vi "Local Client.vi"(6 "timeout (ms) [500]":i32=500, 8 "error in (no error)":errorcluster, 9 "params":variant, 10 "Command in":variant, 11 "Instrument in":refnum<class "Instrument.lvclass">) -> (0 "error out":errorcluster, 1 "Data out":variant, 2 "Command out":string, 3 "Instrument out":refnum<class "Instrument.lvclass">)   [LabVIEW 2019, in "Instrument.lvlib" / "Instrument.lvclass"]
doc: "Send a message to a local Instrument process. This VI is basically a wrapper for Instrument.sendMessageToProcess.vi with a mailbox to receive responses.\n\n<b>Command in</b> is a String. Conversion from Enum needs to be handled before calling this method (Use \"Enum to String.vi\")\n\n<b>Data in</b> is a Variant containing your data payload.\n\n<b>Data out</b> is a Variant."
uses:
  Instrument.lvclass
  c6c297fa-ccfe-4267-9780-fc415f7827cf.vi
  Instrument.sendMessageToProcess (variant).vi
  <vilib>/Utility/Data Type/Get Type Information.vi
  <vilib>/Utility/Data Type/Get Numeric Information.vi
  <userlib>/_OpenG.lib/lvdata/lvdata.llb/Unwrap VVariant__ogtk.vi
panel:
  # "Local Client.vi"
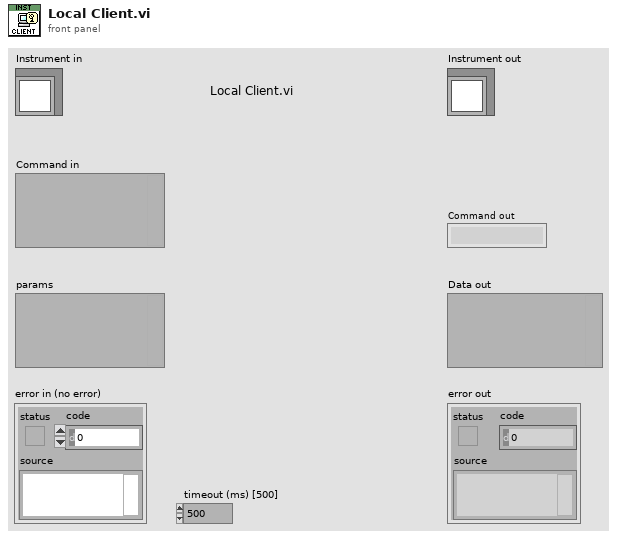
[diagram p1: front panel]
types:
  T1 = typedef "Instrument.lvlib/Instrument.lvclass/PublicEvents--Cluster.ctl" = cluster{"MessageFromProcess":refnum<user-event>}
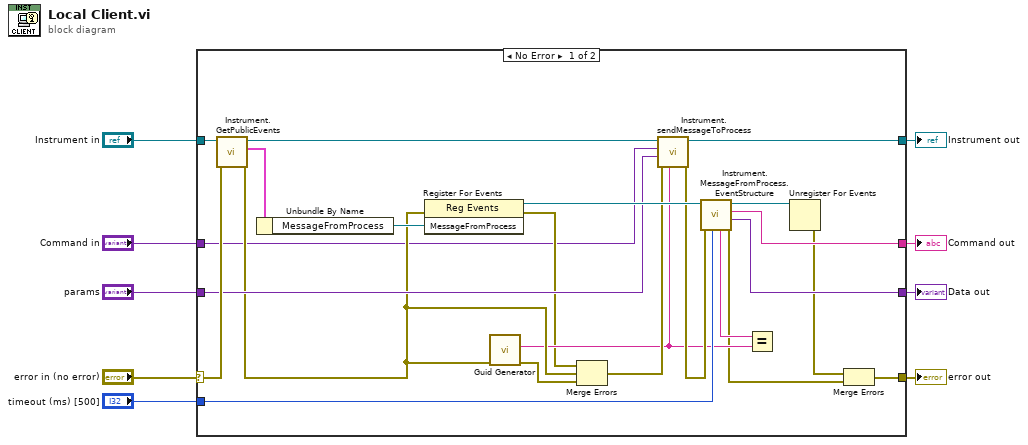
[diagram p0: block diagram]
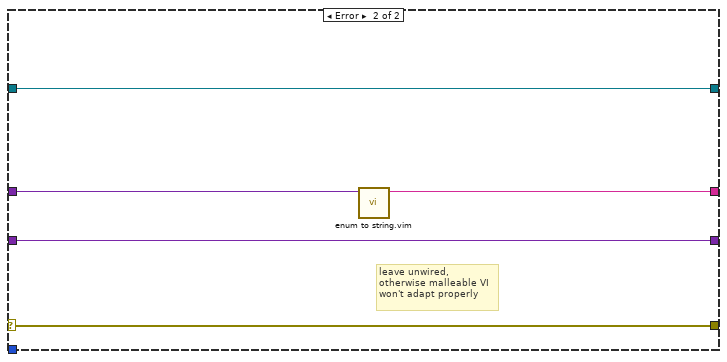
[diagram p2: hidden frame]
diagram:
  n1 = case shown="No Error" "error in (no error)" {
    selector: "error in (no error)" -> [w27 w37]
    tunnel: [w12 w37] -> w8
    tunnel: [w32 w36] -> w6
    tunnel: "Instrument in" -> [w28 w36]
    tunnel: "Command in" -> [w11 w33]
    tunnel: "params" -> [w20 w35]
    tunnel: "timeout (ms) [500]" -> [w22 _]
    tunnel: [w16 w34] -> w3
    tunnel: [w15 w35] -> w2
    frame No Error {
      n2 = call "Instrument.GetPublicEvents.vi"("error in (no error)"=w27, "Instrument"=w28) -> ("error out"=w19:errorcluster, "Instrument Public Events"=w31:T1, "Instrument out"=w10:refnum<class "Instrument.lvclass">)  [unwired: 7 in]
      n3 = Unbundle By Name(w31) -> ("MessageFromProcess"=w30:refnum<user-event>)
      n4 = register-events(error in=w19, w30) -> (reference out=w29:refnum<event-registration>, error out=w17:errorcluster)  [unwired: 1 in]
      n5 = call <vilib>:"Guid Generator.vi"("error in (no error)"=w19) -> ("error out"=w21:errorcluster, "GUID"=w18:string)  [unwired: 9 in]
      n6 = Merge Errors(w17, w19, w21) -> (w25:errorcluster)
      n7 = call-poly "Instrument.sendMessageToProcess.vi"("ID"=w18, "error in (no error)"=w25, "Data"=w20, "Command"=w11, "Instrument"=w10) -> ("error out"=w24:errorcluster, "Instrument out"=w32:refnum<class "Instrument.lvclass">)  [unwired: 5 in]
      n8 = call "Instrument.MessageFromProcess.EventStructure.vi"("timeout (ms) [500]"=w22, "error in (no error)"=w24, "Event Registration Refnum in"=w29) -> ("error out"=w14:errorcluster, "Data"=w15:variant, "Command"=w16:string, "Event Registration Refnum out"=w26:refnum<event-registration>, "ID"=w23:string)  [unwired: 4 in]
      n9 = Equal?(x=w23, y=w18) -> ()  [unwired: 1 out]
      n10 = Unregister For Events(event registration refnum=w26) -> (error out=w13:errorcluster)  [unwired: 1 in]
      n11 = Merge Errors(w13, w14) -> (w12:errorcluster)
    }
    frame Error {
      # "leave unwired,\notherwise malleable VI\nwon't adapt properly"
      n12 = call "enum to string.vim"("enum in"=w33) -> ("string out"=w34:string)  [unwired: 9 in, 1 out]
    }
  }
  "error out" <- w8
  "Instrument out" <- w6
  "Command out" <- w3
  "Data out" <- w2
